vi "Read User Input Entry.vi"(8 "error in":errorcluster, 11 "User Input Enumerator":T2) -> (0 "error out":errorcluster, 3 "Entry":T1)   [LabVIEW 2026, in "ToastNotification.lvlib" / "ToastService.lvclass"]
doc: "Read one entry from a borrowed UserInput enumerator already positioned by a successful MoveNext returning true. Acquire Current, copy its Key and Value strings and close the acquired Current handle on every path. Does not advance, dispose or close the enumerator. Skip on incoming error."
uses:
  ToastService.lvclass
  Reflection DotNet/Callback Object Reference.ctl
  ToastNotification/Argument.ctl
  Reflection DotNet/Reflection DotNet.lvlib
  ToastNotification/ToastNotification.lvlib
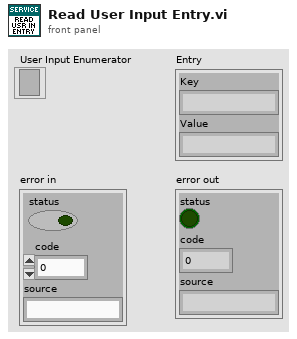
[diagram p1: front panel]
types:
  T1 = typedef "ToastNotification.lvlib/Argument.ctl" = cluster{"Key":string, "Value":string}
  T2 = typedef "ToastNotification.lvlib/Reflection DotNet.lvlib/Callback Object Reference.ctl" = refnum<k24>
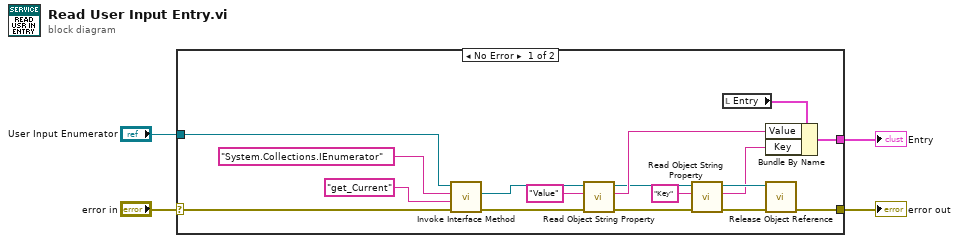
[diagram p0: block diagram]
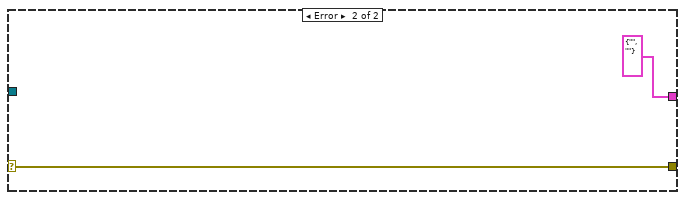
[diagram p2: hidden frame]
diagram:
  n1 = case shown="No Error" "error in" {
    selector: "error in" -> [w16 w22]
    tunnel: "User Input Enumerator" -> [w19 _]
    tunnel: [w21 cluster{"Key":string, "Value":string} {"Key"="", "Value"=""}] -> w3
    tunnel: [w20 w22] -> w4
    frame No Error {
      n2 = call "Invoke Interface Method.vi"("error in"=w16, "method name"="get_Current", "interface name"="System.Collections.IEnumerator", "object in"=w19) -> ("error out"=w13:errorcluster, "value"=w9:T2)  [unwired: 5 in, 1 out]
      n3 = call "Read Object String Property.vi"("error in"=w13, "property name"="Value", "object in"=w9) -> ("error out"=w12:errorcluster, "text"=w10:string, "object out"=w8:T2)  [unwired: 6 in]
      n4 = call "Read Object String Property.vi"("error in"=w12, "property name"="Key", "object in"=w8) -> ("error out"=w11:errorcluster, "text"=w6:string, "object out"=w7:T2)  [unwired: 6 in]
      n5 = local read "Entry"() -> (w5:T1)
      n6 = Bundle By Name(cluster=w5, "Value"=w10, "Key"=w6) -> (w21:T1)
      n7 = call "Release Object Reference.vi"("error in"=w11, "object"=w7) -> ("error out"=w20:errorcluster)  [unwired: 9 in]
    }
    frame Error {
    }
  }
  "Entry" <- w3
  "error out" <- w4
